vi "csb pcap max bytes.vi"(8 "error in (no error)":errorcluster, 11 "n_frames":i32) -> (0 "error out":errorcluster, 3 "function return":i32)   [LabVIEW 2021, in "CANsub_Codec.lvlib"]
doc: "int32_t csb_pcap_max_bytes(int32_t n_frames);"
uses:
  CANsub_Codec.lvlib
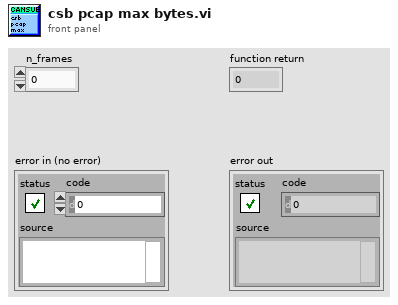
[diagram p1: front panel]
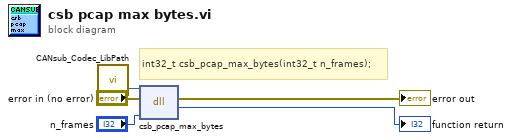
[diagram p0: block diagram]
diagram:
  # "int32_t csb_pcap_max_bytes(int32_t n_frames);"
  n1 = call "CANsub_Codec_LibPath.vi"() -> ("Path"=w1:path)  [unwired: 11 in]
  n2 = dll-call lib="libcansub_codec.*" fn="csb_pcap_max_bytes"(path in=w1, error in="error in (no error)", "n_frames"="n_frames") -> (error out=→"error out":errorcluster, "return type"=→"function return":i32)  [unwired: 2 in, 1 out]
